vi "Safe Setpoints.vi"(11 "Rig Config":T1) -> (3 "setpoints":cluster{"channel":string, "value":dbl}[](array[cluster]))   [LabVIEW 2026]
doc: "Builds a safe setpoint (value 0 clamped into each channel's [min,max]) for every channel of a Rig Config. Used by Stop, E-Stop and Finish to drive the rig to a safe state. Pure function, no error terminals, AF-free."
uses:
  Typedefs/Channel Definition.ctl
  Typedefs/Rig Config.ctl
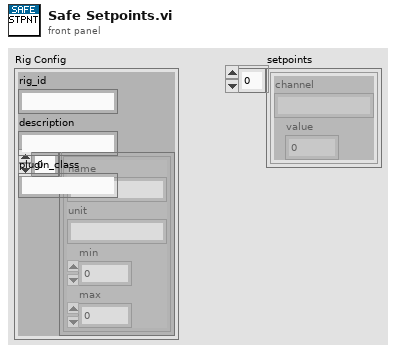
[diagram p1: front panel]
types:
  T1 = typedef "Rig Config.ctl" = cluster{"rig_id":string, "description":string, "plugin_class":string, "channels":T2[]}
  T2 = typedef "Channel Definition.ctl" = cluster{"name":string, "unit":string, "min":dbl, "max":dbl}
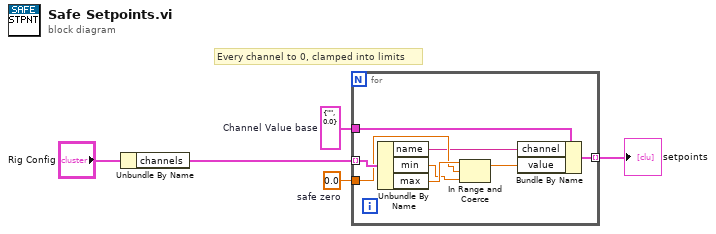
[diagram p0: block diagram]
diagram:
  w2 = cluster{"channel":string, "value":dbl} {"channel"="", "value"=0.0}  # Channel Value base
  w3 = 0.0  # safe zero
  # "Every channel to 0, clamped into limits"
  n1 = Unbundle By Name("Rig Config") -> ("channels"=w4:T2[])
  n2 = for {
    tunnel: w4 -> [w13] mode=indexing
    tunnel: w3 -> [w11]
    tunnel: w2 -> [w7]
    tunnel: [w6] -> w1 mode=indexing
    n3 = Unbundle By Name(w13) -> ("name"=w9:string, "min"=w10:dbl, "max"=w12:dbl)
    n4 = In Range and Coerce(upper limit=w12, x=w11, lower limit=w10) -> (coerced(x)=w8:dbl)  [unwired: 1 out]
    n5 = Bundle By Name(cluster=w7, "channel"=w9, "value"=w8) -> (w6:cluster{"channel":string, "value":dbl})
  }
  "setpoints" <- w1
